vi "Test Insert Entry.vi"(8 "error in":errorcluster, 10 "Work Folder":path, 11 "Test Data Folder":path) -> (0 "error out":errorcluster, 2 "Report":string, 3 "Passed":bool)   [LabVIEW 2026]
doc: "Tests Insert Entry.vi on copies of the schema-v2 sample data, one case folder per case, through Test - Insert Case.vi. Cases: (a) insert in the middle of a finished entry - 3 pieces; (b) at its very start - 2 entries and the original ID deleted; (c) at its very end - 2 entries; (d) covering the whole entry - only the inserted entry; (e) a running original - piece 3 stays running and is returned as Running Entry, also when the inserted End Time is Now; (f) inserted time starting before, ending after or with End = Start, and past Now for a running original - error 5104 and the month file unchanged; (g) an original that runs past midnight into the next month with the insert after midnight - each piece filed in the month of its own start. Per case it checks the error code, the Pieces output, the pieces and the original ID read back from the month files, Running Entry, and whether the month file changed. Pieces are compared as text with tags (orig = the original ID, new = a new ID).\n\nInputs: Test Data Folder; Work Folder; error in. Outputs: Passed; Report; error out.\n\nGenerated by: Claude"
uses:
  Storage/Rows/Time Entry.ctl
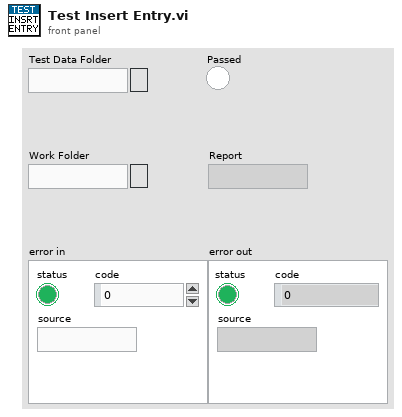
[diagram p1: front panel]
types:
  T1 = typedef "Time Entry.ctl" = cluster{"ID":string, "Project ID":string, "Task ID":string, "Start Time":timestamp, "End Time":timestamp, "Description":string}
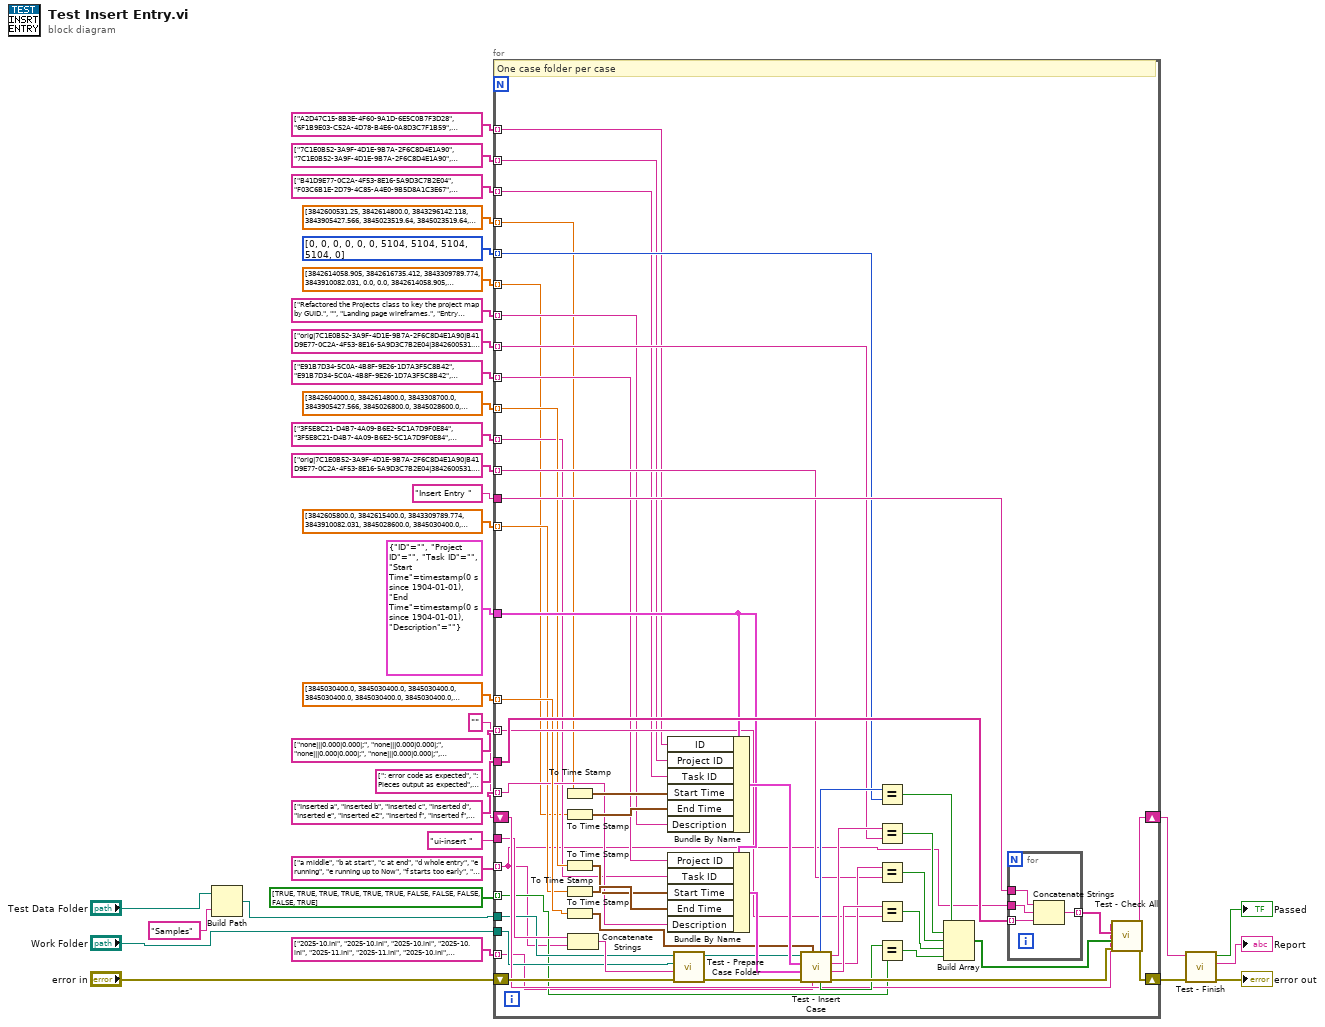
[diagram p0: block diagram]
diagram:
  n1 = Build Path(base path="Test Data Folder", name or relative path="Samples" ("samples")) -> (appended path=w32:path)
  n2 = for {
    tunnel: string[] ["a middle", "b at start", "c at end", "d whole entry", "e running", "e running up to Now", "f starts too early", "f ends too late", "f End equals Start", "f running past Now", "g across midnight and month"] ("case names") -> [w35] mode=indexing
    tunnel: string[] ["A2D47C15-8B3E-4F60-9A1D-6E5C0B7F3D28", "6F1B9E03-C52A-4D78-B4E6-0A8D3C7F1B59", "D80C3A6E-4F17-4B92-8E5D-2C9A1F6B0E73", "39E5B7A2-0D6C-4A1F-9B84-7F2E5D0C3A16", "4C9F1E68-A3D0-4B57-B2E9-6A0C8D5F3B71", "4C9F1E68-A3D0-4B57-B2E9-6A0C8D5F3B71", "A2D47C15-8B3E-4F60-9A1D-6E5C0B7F3D28", "A2D47C15-8B3E-4F60-9A1D-6E5C0B7F3D28", "A2D47C15-8B3E-4F60-9A1D-6E5C0B7F3D28", "4C9F1E68-A3D0-4B57-B2E9-6A0C8D5F3B71", "B5C28F40-7A9D-4E36-A0F1-3D6B9E2C8A47"] ("original IDs") -> [w36] mode=indexing
    tunnel: string[] ["7C1E0B52-3A9F-4D1E-9B7A-2F6C8D4E1A90", "7C1E0B52-3A9F-4D1E-9B7A-2F6C8D4E1A90", "2A6F4C18-9D3B-4E7A-A1C5-8B0E6D2F4A73", "2A6F4C18-9D3B-4E7A-A1C5-8B0E6D2F4A73", "7C1E0B52-3A9F-4D1E-9B7A-2F6C8D4E1A90", "7C1E0B52-3A9F-4D1E-9B7A-2F6C8D4E1A90", "7C1E0B52-3A9F-4D1E-9B7A-2F6C8D4E1A90", "7C1E0B52-3A9F-4D1E-9B7A-2F6C8D4E1A90", "7C1E0B52-3A9F-4D1E-9B7A-2F6C8D4E1A90", "7C1E0B52-3A9F-4D1E-9B7A-2F6C8D4E1A90", "7C1E0B52-3A9F-4D1E-9B7A-2F6C8D4E1A90"] ("original project IDs") -> [w37] mode=indexing
    tunnel: string[] ["B41D9E77-0C2A-4F53-8E16-5A9D3C7B2E04", "F03C6B1E-2D79-4C85-A4E0-9B5D8A1C3E67", "8E2D5A47-1B6C-4F90-8D3A-7C4B0E9F2A16", "C7A40F9B-6E31-4B2D-8C57-2A9D0E4F6B38", "5D8A2C90-7E14-4A6B-B3F9-0C6E1A4D7B25", "5D8A2C90-7E14-4A6B-B3F9-0C6E1A4D7B25", "B41D9E77-0C2A-4F53-8E16-5A9D3C7B2E04", "B41D9E77-0C2A-4F53-8E16-5A9D3C7B2E04", "B41D9E77-0C2A-4F53-8E16-5A9D3C7B2E04", "5D8A2C90-7E14-4A6B-B3F9-0C6E1A4D7B25", "B41D9E77-0C2A-4F53-8E16-5A9D3C7B2E04"] ("original task IDs") -> [w38] mode=indexing
    tunnel: dbl[] [3842600531.25, 3842614800.0, 3843296142.118, 3843905427.566, 3845023519.64, 3845023519.64, 3842600531.25, 3842600531.25, 3842600531.25, 3845023519.64, 3844795205.332] ("original starts") -> [w39] mode=indexing
    tunnel: dbl[] [3842614058.905, 3842616735.412, 3843309789.774, 3843910082.031, 0.0, 0.0, 3842614058.905, 3842614058.905, 3842614058.905, 0.0, 3844804367.019] ("original ends") -> [w40] mode=indexing
    tunnel: string[] ["Refactored the Projects class to key the project map by GUID.", "", "Landing page wireframes.", "Entry against a task that has since been made inactive.", "Still running: an empty End Time marks the active entry.", "Still running: an empty End Time marks the active entry.", "Refactored the Projects class to key the project map by GUID.", "Refactored the Projects class to key the project map by GUID.", "Refactored the Projects class to key the project map by GUID.", "Still running: an empty End Time marks the active entry.", "Runs past midnight into November; filed here because the month file is chosen by Start Time."] ("original descriptions") -> [w41] mode=indexing
    tunnel: string[] ["E91B7D34-5C0A-4B8F-9E26-1D7A3F5C8B42", "E91B7D34-5C0A-4B8F-9E26-1D7A3F5C8B42", "E91B7D34-5C0A-4B8F-9E26-1D7A3F5C8B42", "E91B7D34-5C0A-4B8F-9E26-1D7A3F5C8B42", "E91B7D34-5C0A-4B8F-9E26-1D7A3F5C8B42", "E91B7D34-5C0A-4B8F-9E26-1D7A3F5C8B42", "E91B7D34-5C0A-4B8F-9E26-1D7A3F5C8B42", "E91B7D34-5C0A-4B8F-9E26-1D7A3F5C8B42", "E91B7D34-5C0A-4B8F-9E26-1D7A3F5C8B42", "E91B7D34-5C0A-4B8F-9E26-1D7A3F5C8B42", "E91B7D34-5C0A-4B8F-9E26-1D7A3F5C8B42"] ("inserted project IDs") -> [w42] mode=indexing
    tunnel: string[] ["3F5E8C21-D4B7-4A09-B6E2-5C1A7D9F0E84", "3F5E8C21-D4B7-4A09-B6E2-5C1A7D9F0E84", "3F5E8C21-D4B7-4A09-B6E2-5C1A7D9F0E84", "3F5E8C21-D4B7-4A09-B6E2-5C1A7D9F0E84", "3F5E8C21-D4B7-4A09-B6E2-5C1A7D9F0E84", "3F5E8C21-D4B7-4A09-B6E2-5C1A7D9F0E84", "3F5E8C21-D4B7-4A09-B6E2-5C1A7D9F0E84", "3F5E8C21-D4B7-4A09-B6E2-5C1A7D9F0E84", "3F5E8C21-D4B7-4A09-B6E2-5C1A7D9F0E84", "3F5E8C21-D4B7-4A09-B6E2-5C1A7D9F0E84", "3F5E8C21-D4B7-4A09-B6E2-5C1A7D9F0E84"] ("inserted task IDs") -> [w43] mode=indexing
    tunnel: dbl[] [3842604000.0, 3842614800.0, 3843308700.0, 3843905427.566, 3845026800.0, 3845028600.0, 3842600400.0, 3842611200.0, 3842605800.0, 3845028600.0, 3844800030.0] ("inserted starts") -> [w44] mode=indexing
    tunnel: dbl[] [3842605800.0, 3842615400.0, 3843309789.774, 3843910082.031, 3845028600.0, 3845030400.0, 3842604000.0, 3842614800.0, 3842605800.0, 3845032200.0, 3844801800.0] ("inserted ends") -> [w45] mode=indexing
    tunnel: string[] ["Inserted a", "Inserted b", "Inserted c", "Inserted d", "Inserted e", "Inserted e2", "Inserted f", "Inserted f", "Inserted f", "Inserted f", "Inserted g"] ("inserted descriptions") -> [w46] mode=indexing
    tunnel: dbl[] [3845030400.0, 3845030400.0, 3845030400.0, 3845030400.0, 3845030400.0, 3845030400.0, 3845030400.0, 3845030400.0, 3845030400.0, 3845030400.0, 3845030400.0] ("nows") -> [w47] mode=indexing
    tunnel: string[] ["2025-10.ini", "2025-10.ini", "2025-10.ini", "2025-10.ini", "2025-11.ini", "2025-11.ini", "2025-10.ini", "2025-10.ini", "2025-10.ini", "2025-11.ini", "2025-10.ini"] ("month files") -> [w48] mode=indexing
    tunnel: i32[] [0, 0, 0, 0, 0, 0, 5104, 5104, 5104, 5104, 0] ("expected codes") -> [w49] mode=indexing
    tunnel: string[] ["orig|7C1E0B52-3A9F-4D1E-9B7A-2F6C8D4E1A90|B41D9E77-0C2A-4F53-8E16-5A9D3C7B2E04|3842600531.250|3842604000.000|Refactored the Projects class to key the project map by GUID.;new|E91B7D34-5C0A-4B8F-9E26-1D7A3F5C8B42|3F5E8C21-D4B7-4A09-B6E2-5C1A7D9F0E84|3842604000.000|3842605800.000|Inserted a;new|7C1E0B52-3A9F-4D1E-9B7A-2F6C8D4E1A90|B41D9E77-0C2A-4F53-8E16-5A9D3C7B2E04|3842605800.000|3842614058.905|;", "new|E91B7D34-5C0A-4B8F-9E26-1D7A3F5C8B42|3F5E8C21-D4B7-4A09-B6E2-5C1A7D9F0E84|3842614800.000|3842615400.000|Inserted b;new|7C1E0B52-3A9F-4D1E-9B7A-2F6C8D4E1A90|F03C6B1E-2D79-4C85-A4E0-9B5D8A1C3E67|3842615400.000|3842616735.412|;", "orig|2A6F4C18-9D3B-4E7A-A1C5-8B0E6D2F4A73|8E2D5A47-1B6C-4F90-8D3A-7C4B0E9F2A16|3843296142.118|3843308700.000|Landing page wireframes.;new|E91B7D34-5C0A-4B8F-9E26-1D7A3F5C8B42|3F5E8C21-D4B7-4A09-B6E2-5C1A7D9F0E84|3843308700.000|3843309789.774|Inserted c;", "new|E91B7D34-5C0A-4B8F-9E26-1D7A3F5C8B42|3F5E8C21-D4B7-4A09-B6E2-5C1A7D9F0E84|3843905427.566|3843910082.031|Inserted d;", "orig|7C1E0B52-3A9F-4D1E-9B7A-2F6C8D4E1A90|5D8A2C90-7E14-4A6B-B3F9-0C6E1A4D7B25|3845023519.640|3845026800.000|Still running: an empty End Time marks the active entry.;new|E91B7D34-5C0A-4B8F-9E26-1D7A3F5C8B42|3F5E8C21-D4B7-4A09-B6E2-5C1A7D9F0E84|3845026800.000|3845028600.000|Inserted e;new|7C1E0B52-3A9F-4D1E-9B7A-2F6C8D4E1A90|5D8A2C90-7E14-4A6B-B3F9-0C6E1A4D7B25|3845028600.000|0.000|;", "orig|7C1E0B52-3A9F-4D1E-9B7A-2F6C8D4E1A90|5D8A2C90-7E14-4A6B-B3F9-0C6E1A4D7B25|3845023519.640|3845028600.000|Still running: an empty End Time marks the active entry.;new|E91B7D34-5C0A-4B8F-9E26-1D7A3F5C8B42|3F5E8C21-D4B7-4A09-B6E2-5C1A7D9F0E84|3845028600.000|3845030400.000|Inserted e2;new|7C1E0B52-3A9F-4D1E-9B7A-2F6C8D4E1A90|5D8A2C90-7E14-4A6B-B3F9-0C6E1A4D7B25|3845030400.000|0.000|;", "", "", "", "", "orig|7C1E0B52-3A9F-4D1E-9B7A-2F6C8D4E1A90|B41D9E77-0C2A-4F53-8E16-5A9D3C7B2E04|3844795205.332|3844800030.000|Runs past midnight into November; filed here because the month file is chosen by Start Time.;new|E91B7D34-5C0A-4B8F-9E26-1D7A3F5C8B42|3F5E8C21-D4B7-4A09-B6E2-5C1A7D9F0E84|3844800030.000|3844801800.000|Inserted g;new|7C1E0B52-3A9F-4D1E-9B7A-2F6C8D4E1A90|B41D9E77-0C2A-4F53-8E16-5A9D3C7B2E04|3844801800.000|3844804367.019|;"] ("expected pieces") -> [w50] mode=indexing
    tunnel: string[] ["orig|7C1E0B52-3A9F-4D1E-9B7A-2F6C8D4E1A90|B41D9E77-0C2A-4F53-8E16-5A9D3C7B2E04|3842600531.250|3842604000.000|Refactored the Projects class to key the project map by GUID.;new|E91B7D34-5C0A-4B8F-9E26-1D7A3F5C8B42|3F5E8C21-D4B7-4A09-B6E2-5C1A7D9F0E84|3842604000.000|3842605800.000|Inserted a;new|7C1E0B52-3A9F-4D1E-9B7A-2F6C8D4E1A90|B41D9E77-0C2A-4F53-8E16-5A9D3C7B2E04|3842605800.000|3842614058.905|;orig|7C1E0B52-3A9F-4D1E-9B7A-2F6C8D4E1A90|B41D9E77-0C2A-4F53-8E16-5A9D3C7B2E04|3842600531.250|3842604000.000|Refactored the Projects class to key the project map by GUID.;", "new|E91B7D34-5C0A-4B8F-9E26-1D7A3F5C8B42|3F5E8C21-D4B7-4A09-B6E2-5C1A7D9F0E84|3842614800.000|3842615400.000|Inserted b;new|7C1E0B52-3A9F-4D1E-9B7A-2F6C8D4E1A90|F03C6B1E-2D79-4C85-A4E0-9B5D8A1C3E67|3842615400.000|3842616735.412|;none|||0.000|0.000|;", "orig|2A6F4C18-9D3B-4E7A-A1C5-8B0E6D2F4A73|8E2D5A47-1B6C-4F90-8D3A-7C4B0E9F2A16|3843296142.118|3843308700.000|Landing page wireframes.;new|E91B7D34-5C0A-4B8F-9E26-1D7A3F5C8B42|3F5E8C21-D4B7-4A09-B6E2-5C1A7D9F0E84|3843308700.000|3843309789.774|Inserted c;orig|2A6F4C18-9D3B-4E7A-A1C5-8B0E6D2F4A73|8E2D5A47-1B6C-4F90-8D3A-7C4B0E9F2A16|3843296142.118|3843308700.000|Landing page wireframes.;", "new|E91B7D34-5C0A-4B8F-9E26-1D7A3F5C8B42|3F5E8C21-D4B7-4A09-B6E2-5C1A7D9F0E84|3843905427.566|3843910082.031|Inserted d;none|||0.000|0.000|;", "orig|7C1E0B52-3A9F-4D1E-9B7A-2F6C8D4E1A90|5D8A2C90-7E14-4A6B-B3F9-0C6E1A4D7B25|3845023519.640|3845026800.000|Still running: an empty End Time marks the active entry.;new|E91B7D34-5C0A-4B8F-9E26-1D7A3F5C8B42|3F5E8C21-D4B7-4A09-B6E2-5C1A7D9F0E84|3845026800.000|3845028600.000|Inserted e;new|7C1E0B52-3A9F-4D1E-9B7A-2F6C8D4E1A90|5D8A2C90-7E14-4A6B-B3F9-0C6E1A4D7B25|3845028600.000|0.000|;orig|7C1E0B52-3A9F-4D1E-9B7A-2F6C8D4E1A90|5D8A2C90-7E14-4A6B-B3F9-0C6E1A4D7B25|3845023519.640|3845026800.000|Still running: an empty End Time marks the active entry.;", "orig|7C1E0B52-3A9F-4D1E-9B7A-2F6C8D4E1A90|5D8A2C90-7E14-4A6B-B3F9-0C6E1A4D7B25|3845023519.640|3845028600.000|Still running: an empty End Time marks the active entry.;new|E91B7D34-5C0A-4B8F-9E26-1D7A3F5C8B42|3F5E8C21-D4B7-4A09-B6E2-5C1A7D9F0E84|3845028600.000|3845030400.000|Inserted e2;new|7C1E0B52-3A9F-4D1E-9B7A-2F6C8D4E1A90|5D8A2C90-7E14-4A6B-B3F9-0C6E1A4D7B25|3845030400.000|0.000|;orig|7C1E0B52-3A9F-4D1E-9B7A-2F6C8D4E1A90|5D8A2C90-7E14-4A6B-B3F9-0C6E1A4D7B25|3845023519.640|3845028600.000|Still running: an empty End Time marks the active entry.;", "orig|7C1E0B52-3A9F-4D1E-9B7A-2F6C8D4E1A90|B41D9E77-0C2A-4F53-8E16-5A9D3C7B2E04|3842600531.250|3842614058.905|Refactored the Projects class to key the project map by GUID.;", "orig|7C1E0B52-3A9F-4D1E-9B7A-2F6C8D4E1A90|B41D9E77-0C2A-4F53-8E16-5A9D3C7B2E04|3842600531.250|3842614058.905|Refactored the Projects class to key the project map by GUID.;", "orig|7C1E0B52-3A9F-4D1E-9B7A-2F6C8D4E1A90|B41D9E77-0C2A-4F53-8E16-5A9D3C7B2E04|3842600531.250|3842614058.905|Refactored the Projects class to key the project map by GUID.;", "orig|7C1E0B52-3A9F-4D1E-9B7A-2F6C8D4E1A90|5D8A2C90-7E14-4A6B-B3F9-0C6E1A4D7B25|3845023519.640|0.000|Still running: an empty End Time marks the active entry.;", "orig|7C1E0B52-3A9F-4D1E-9B7A-2F6C8D4E1A90|B41D9E77-0C2A-4F53-8E16-5A9D3C7B2E04|3844795205.332|3844800030.000|Runs past midnight into November; filed here because the month file is chosen by Start Time.;new|E91B7D34-5C0A-4B8F-9E26-1D7A3F5C8B42|3F5E8C21-D4B7-4A09-B6E2-5C1A7D9F0E84|3844800030.000|3844801800.000|Inserted g;new|7C1E0B52-3A9F-4D1E-9B7A-2F6C8D4E1A90|B41D9E77-0C2A-4F53-8E16-5A9D3C7B2E04|3844801800.000|3844804367.019|;orig|7C1E0B52-3A9F-4D1E-9B7A-2F6C8D4E1A90|B41D9E77-0C2A-4F53-8E16-5A9D3C7B2E04|3844795205.332|3844800030.000|Runs past midnight into November; filed here because the month file is chosen by Start Time.;"] ("expected reread") -> [w51] mode=indexing
    tunnel: string[] ["none|||0.000|0.000|;", "none|||0.000|0.000|;", "none|||0.000|0.000|;", "none|||0.000|0.000|;", "new|7C1E0B52-3A9F-4D1E-9B7A-2F6C8D4E1A90|5D8A2C90-7E14-4A6B-B3F9-0C6E1A4D7B25|3845028600.000|0.000|;", "new|7C1E0B52-3A9F-4D1E-9B7A-2F6C8D4E1A90|5D8A2C90-7E14-4A6B-B3F9-0C6E1A4D7B25|3845030400.000|0.000|;", "none|||0.000|0.000|;", "none|||0.000|0.000|;", "none|||0.000|0.000|;", "none|||0.000|0.000|;", "none|||0.000|0.000|;"] ("expected running") -> [w52] mode=indexing
    tunnel: bool[] [TRUE, TRUE, TRUE, TRUE, TRUE, TRUE, FALSE, FALSE, FALSE, FALSE, TRUE] ("expected changed") -> [w53] mode=indexing
    tunnel: "Work Folder" -> [w54]
    tunnel: T1 {"ID"="", "Project ID"="", "Task ID"="", "Start Time"=timestamp(0 s since 1904-01-01), "End Time"=timestamp(0 s since 1904-01-01), "Description"=""} ("entry template") -> [w56]
    tunnel: string[] [": error code as expected", ": Pieces output as expected", ": pieces and original ID read back from the month files", ": Running Entry as expected", ": month file changed only when something was written"] ("check suffixes") -> [w57]
    tunnel: "Insert Entry " ("check prefix") -> [w58]
    tunnel: "ui-insert " ("case prefix") -> [w59]
    shift-right: [w61] -> w33
    shift-left: "" ("empty report") -> [w60]
    shift-right: [w63] -> w34
    shift-left: "error in" -> [w62]
    tunnel: w32 -> [w55]
    # "One case folder per case"
    n3 = To Time Stamp(1:w39) -> (0:w67:timestamp)
    n4 = To Time Stamp(1:w40) -> (0:w68:timestamp)
    n5 = To Time Stamp(1:w44) -> (0:w69:timestamp)
    n6 = To Time Stamp(1:w45) -> (0:w70:timestamp)
    n7 = To Time Stamp(1:w47) -> (0:w71:timestamp)
    n8 = Concatenate Strings(w59, w35) -> (w64:string)
    n9 = Bundle By Name(cluster=w56, "ID"=w36, "Project ID"=w37, "Task ID"=w38, "Start Time"=w67, "End Time"=w68, "Description"=w41) -> (w72:T1)
    n10 = Bundle By Name(cluster=w56, "Project ID"=w42, "Task ID"=w43, "Start Time"=w69, "End Time"=w70, "Description"=w46) -> (w73:T1)
    n11 = call "Test - Prepare Case Folder.vi"("error in (no error)"=w62, "Case Name"=w64, "Work Folder"=w54, "Source Folder"=w55) -> ("error out"=w65:errorcluster, "Case Folder"=w66:path)  [unwired: 6 in]
    n12 = call "Test - Insert Case.vi"("Month File"=w48, "Now"=w71, "error in"=w65, "Inserted Entry"=w73, "Original Entry"=w72, "Case Folder"=w66) -> ("error out"=w79:errorcluster, "Running Text"=w76:string, "Reread Text"=w75:string, "Pieces Text"=w74:string, "Month File Changed?"=w78:bool, "Insert Error Code"=w77:i32)
    n13 = Equal?(x=w77, y=w49) -> (x = y?=w80:bool)
    n14 = Equal?(x=w74, y=w50) -> (x = y?=w81:bool)
    n15 = Equal?(x=w75, y=w51) -> (x = y?=w82:bool)
    n16 = Equal?(x=w76, y=w52) -> (x = y?=w83:bool)
    n17 = Equal?(x=w78, y=w53) -> (x = y?=w84:bool)
    n18 = Build Array(w80, w81, w82, w83, w84) -> (w85:bool[])
    n19 = for {
      tunnel: w57 -> [w87] mode=indexing
      tunnel: w35 -> [w88]
      tunnel: w58 -> [w89]
      tunnel: [w90] -> w86 mode=indexing
      n20 = Concatenate Strings(w89, w88, w87) -> (w90:string)
    }
    n21 = call "Test - Check All.vi"("error in"=w79, "Conditions"=w85, "Check Names"=w86, "Report in"=w60) -> ("error out"=w63:errorcluster, "Report out"=w61:string)  [unwired: 6 in]
  }
  n22 = call "Test - Finish.vi"("error in (no error)"=w34, "Report"=w33) -> ("error out"=→"error out":errorcluster, "Report out"=→"Report":string, "Passed"=→"Passed":bool)  [unwired: 7 in]
